vi "Update Market Mood.vi"(11 "market":T1) -> (3 "market out":T1)   [LabVIEW 2020, in "Full Featured MCP Server.lvlib"]
doc: "Lets the mood of the market drift for one second. mood swings slowly around zero and pulls all stocks with it (each by its beta), every sector has a mood of its own, and tension is the nervousness of the whole market: it jumps up now and then and calms down again, which gives quiet and nervous phases."
uses:
  Full Featured MCP Server.lvlib
  Market State.ctl
  News Item.ctl
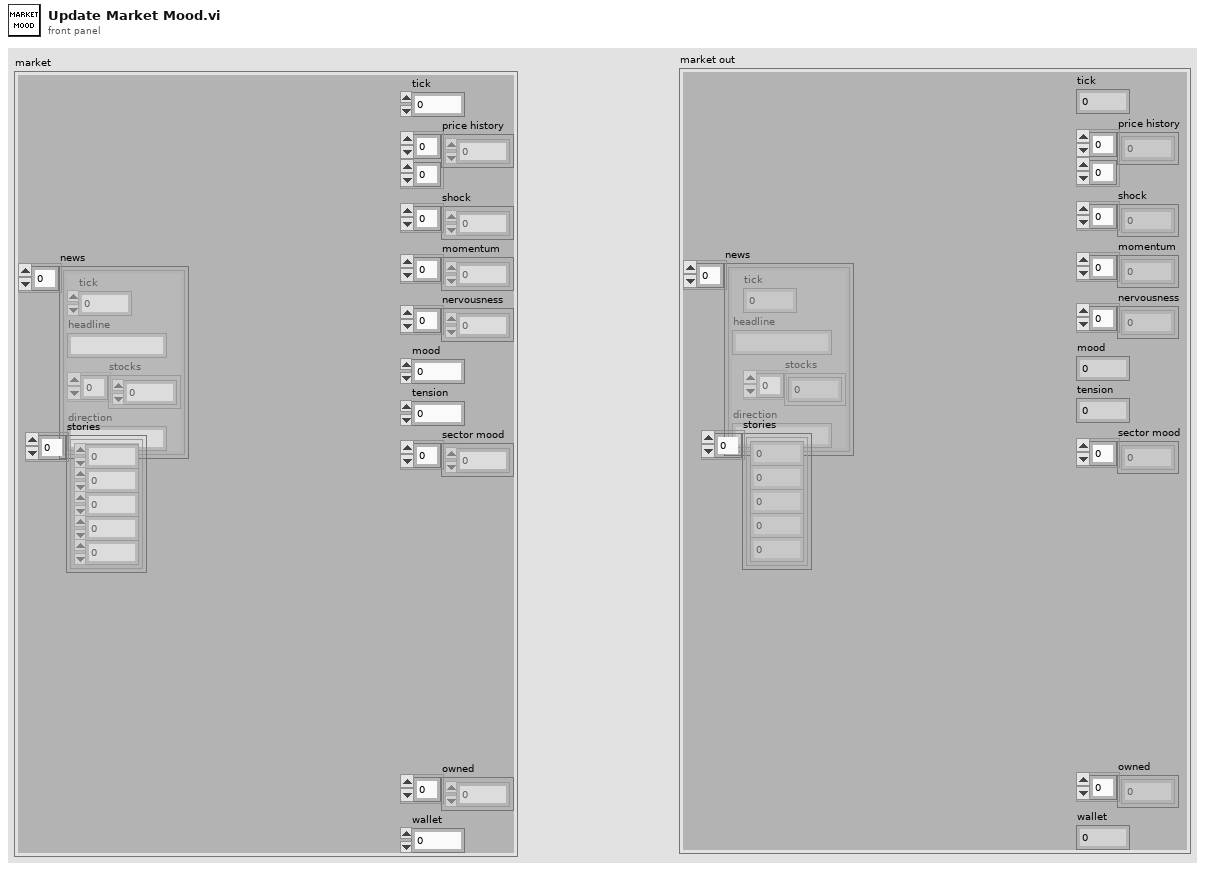
[diagram p1: front panel]
types:
  T1 = typedef "Full Featured MCP Server.lvlib/Market State.ctl" = cluster{"tick":i32, "price history":dbl[][], "shock":dbl[], "momentum":dbl[], "nervousness":dbl[], "mood":dbl, "tension":dbl, "sector mood":dbl[], "news":T2[], "stories":cluster{"arc":i32, "step":i32, "due":i32, "stock":i32, "other":i32}[], "owned":i32[], "wallet":dbl}
  T2 = typedef "Full Featured MCP Server.lvlib/News Item.ctl" = cluster{"tick":i32, "headline":string, "stocks":i32[], "direction":string}
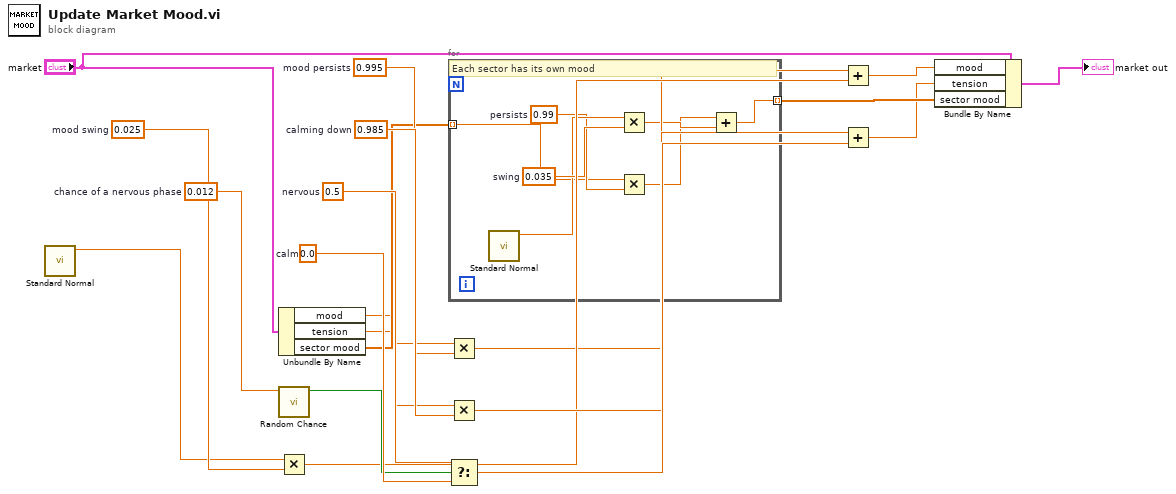
[diagram p0: block diagram]
diagram:
  w16 = 0.0  # calm
  w15 = 0.5  # nervous
  w13 = 0.985  # calming down
  w11 = 0.012  # chance of a nervous phase
  w8 = 0.025  # mood swing
  w5 = 0.995  # mood persists
  n1 = call "Standard Normal.vi"() -> ("number"=w7:dbl)  [unwired: 11 in]
  n2 = Unbundle By Name("market") -> ("mood"=w2:dbl, "tension"=w3:dbl, "sector mood"=w4:dbl[])
  n3 = call "Random Chance.vi"("probability"=w11) -> ("happened?"=w12:bool)  [unwired: 10 in]
  n4 = Multiply(x=w7, y=w8) -> (x*y=w9:dbl)
  n5 = for {
    tunnel: w4 -> [w21] mode=indexing
    tunnel: [w27] -> w19 mode=indexing
    w25 = 0.035  # swing
    w22 = 0.99  # persists
    # "Each sector has its own mood"
    n6 = call "Standard Normal.vi"() -> ("number"=w24:dbl)  [unwired: 11 in]
    n7 = Multiply(x=w24, y=w25) -> (x*y=w26:dbl)
    n8 = Multiply(x=w21, y=w22) -> (x*y=w23:dbl)
    n9 = Add(x=w23, y=w26) -> (x+y=w27:dbl)
  }
  n10 = Multiply(x=w2, y=w5) -> (x*y=w6:dbl)
  n11 = Multiply(x=w3, y=w13) -> (x*y=w14:dbl)
  n12 = Select(t=w15, s=w12, f=w16) -> (s? t:f=w17:dbl)
  n13 = Add(x=w6, y=w9) -> (x+y=w10:dbl)
  n14 = Add(x=w14, y=w17) -> (x+y=w18:dbl)
  n15 = Bundle By Name(cluster="market", "mood"=w10, "tension"=w18, "sector mood"=w19) -> (→"market out":T1)
